vi "Water Tunnel Front Panel.vi"() -> ()   [LabVIEW 2019, in "Results.lvlib" / "Water Tunnel Results.lvclass"]
uses:
  Water Tunnel Results.lvclass
  Water Tunnel Results.lvclass/Water Tunnel Results.ctl
  Test Stands/Water Tunnel/Water Tunnel Test Stand.lvclass
panel:
  out "Water Flow Slide":dbl(slide) scale=0.0..100.0
  out "Wing Test":bool caption="Test"
  out "Wing Home":bool caption="Home"
  out "3-D Velocity":cluster{"Vx":dbl, "Vy":dbl, "Vz":dbl}
  out "Water flow":dbl format="%#.2f"
  out "Wing Angle of Attack":dbl(knob) scale=-45.0..45.0
  out "Probe depth":dbl(slide) scale=-100.0..100.0
  in  "Probe Z-Axis (Depth)":dbl
  in  "Wing Angle of Attack":dbl
  in  "Wing Test Position":bool
  in  "Wing Home Position":bool
  out "Wing Aligned?":bool=TRUE caption="Wing"
  out "Probe Aligned?":bool=TRUE caption="Probe"
  in  "Trav SetP":cluster{"Wx":dbl, "Wz":dbl, "Wa":dbl, "Pz":dbl}
  in  "Trav Probe Set?":bool caption="Probe Traverse"
  in  "Trav Wing Set?":bool caption="Wing Traverse"
  in  "Pump Load":dbl caption="Pump Load, %" step=10.0 format="%#.2f"
  out "p8":dbl format="%#.2f"
  out "p7":dbl format="%#.2f"
  out "p6":dbl format="%#.2f"
  out "p4":dbl format="%#.2f"
  out "p2":dbl format="%#.2f"
  out "p1":dbl format="%#.2f"
  out "p3":dbl format="%#.2f"
  out "p5":dbl format="%#.2f"
  out "Angle U":dbl format="%#.4f"
  out "Angle":dbl caption="Pitch" format="%#.2f"
  out "Data":waveform(dbl)[](graph) caption="Pressures"
  # "V"
  # "deg"
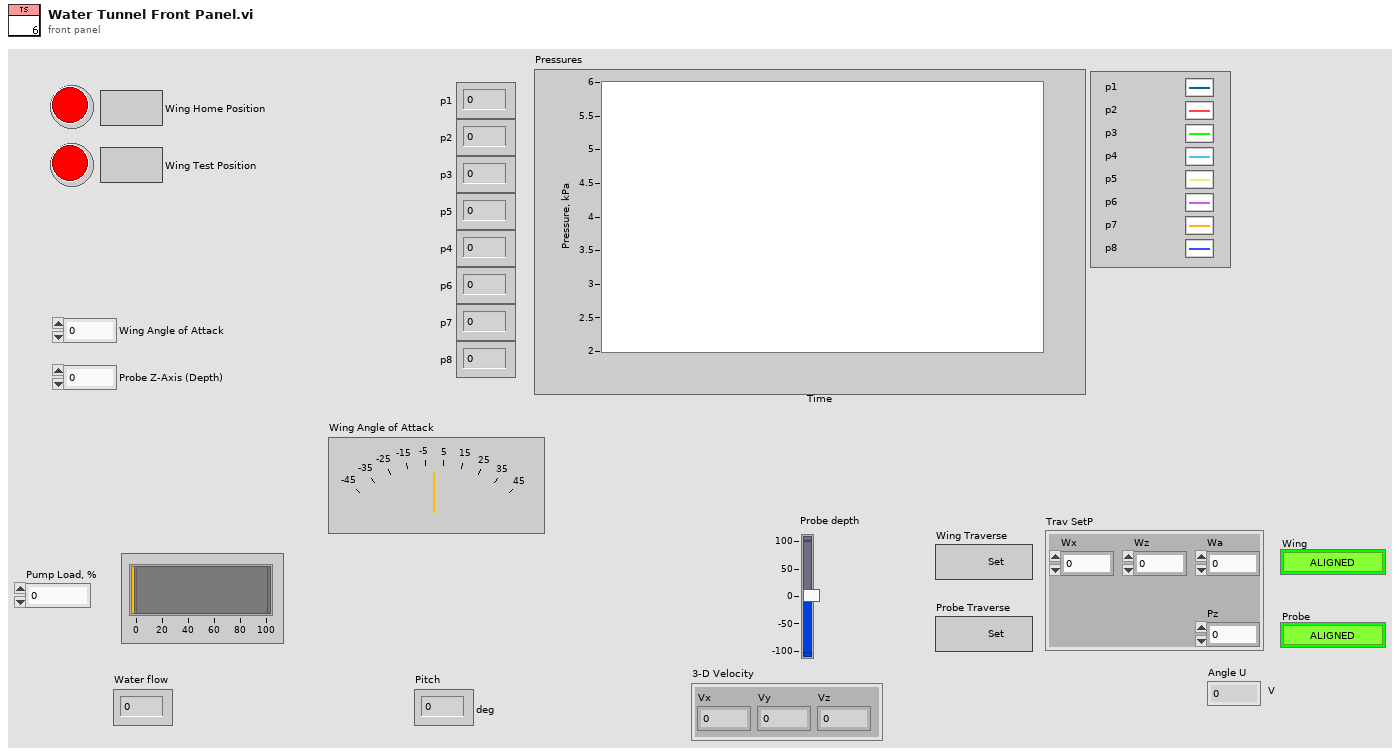
[diagram p1: front panel]
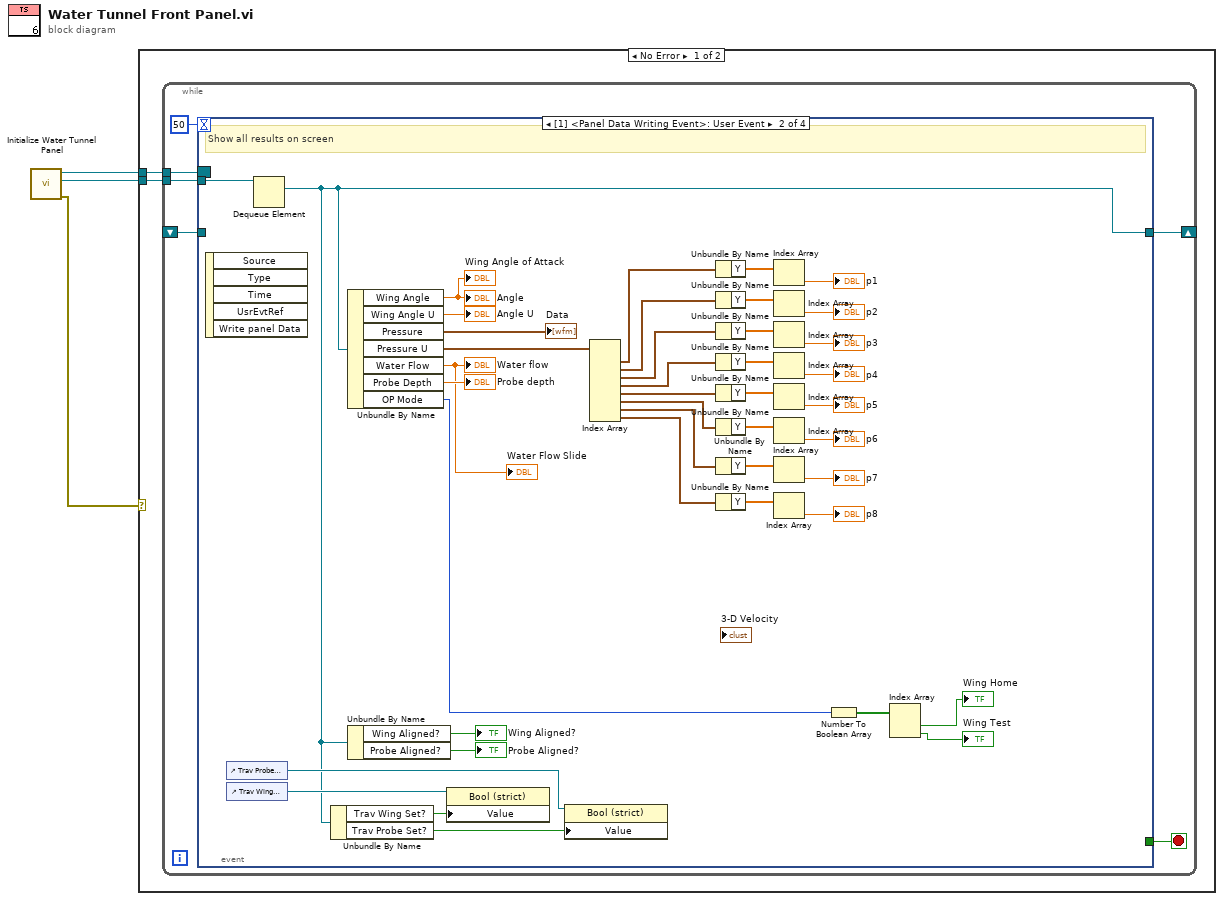
[diagram p0: block diagram]
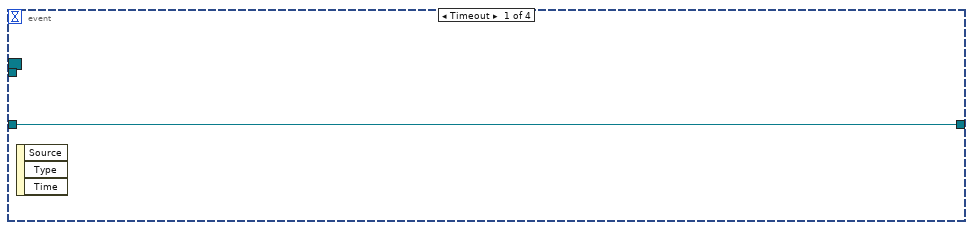
[diagram p2: hidden frame]
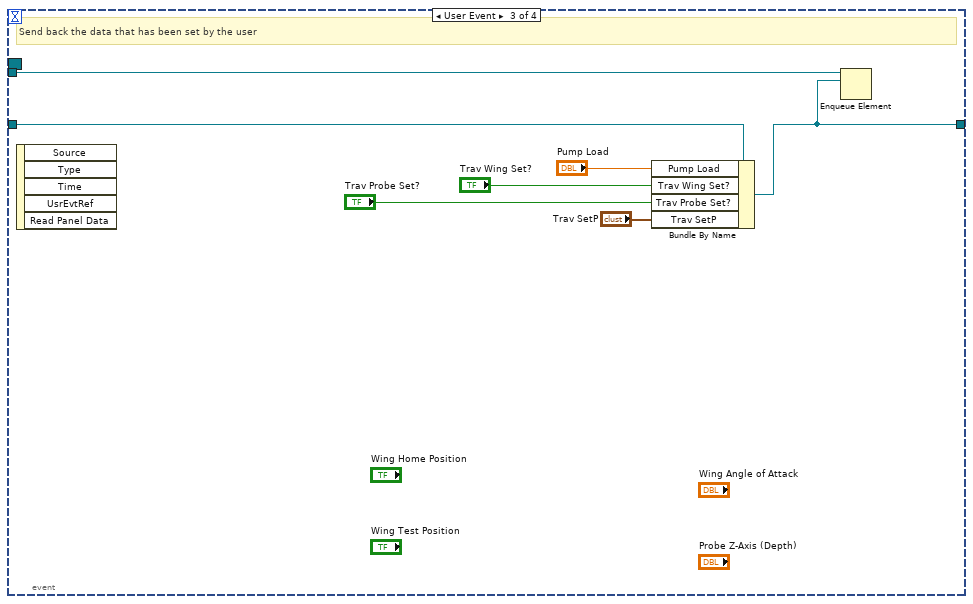
[diagram p3: hidden frame]
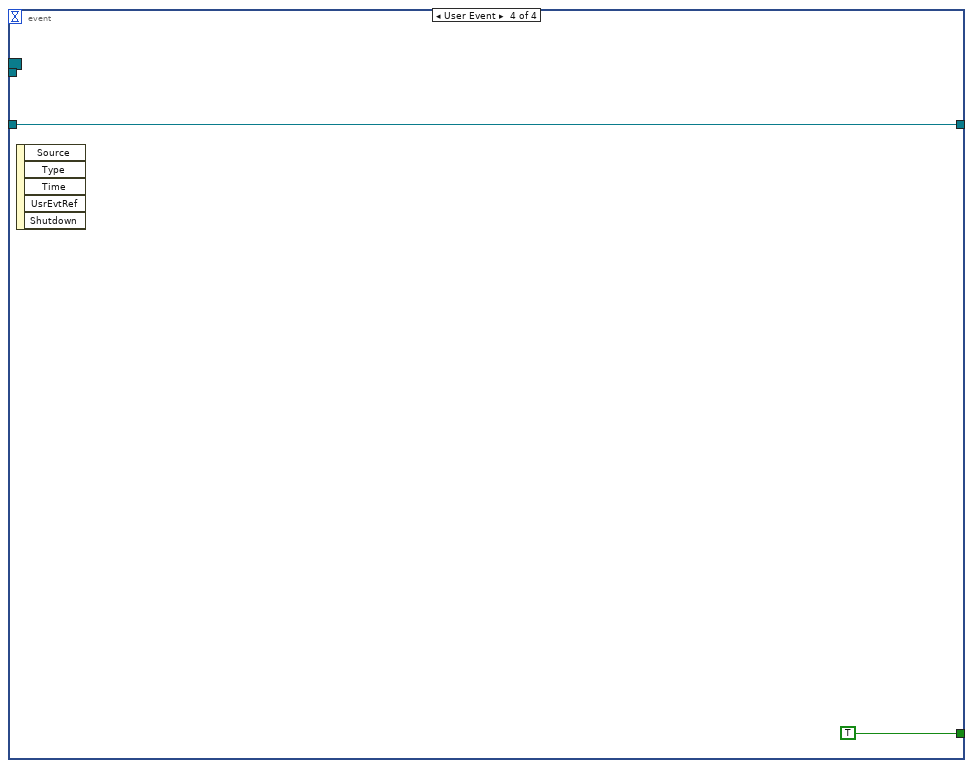
[diagram p4: hidden frame]
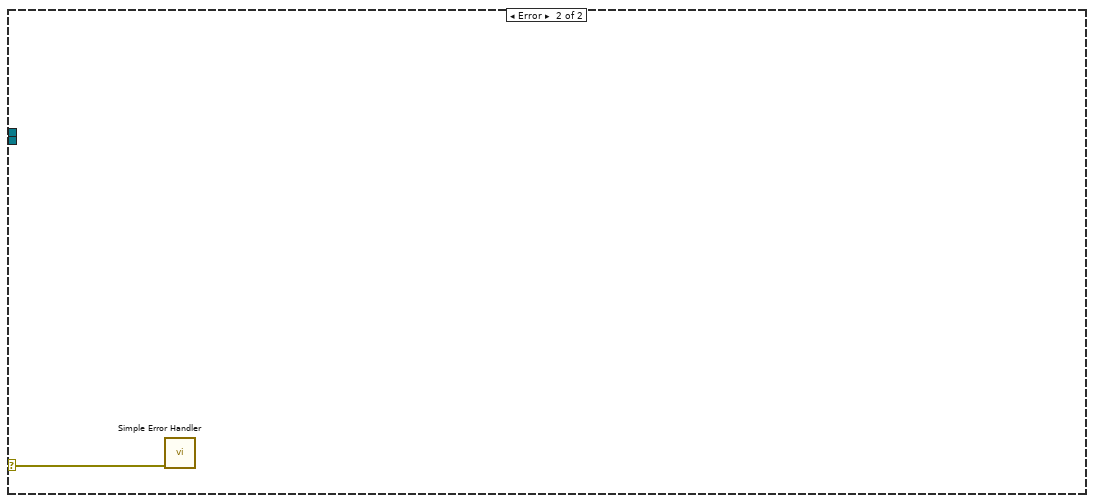
[diagram p5: hidden frame]
diagram:
  n1 = call "Initialize Water Tunnel Panel.vi"() -> ("error out"=w1:errorcluster, "Water Tunnel Results queue out"=w2:refnum<queue>, "Event Registration Refnum"=w3:refnum<event-registration>)  [unwired: 9 in]
  n2 = case shown="No Error" w1 {
    selector: w1 -> [_ w64]
    tunnel: w3 -> [w5 _]
    tunnel: w2 -> [w4 _]
    frame No Error {
      n3 = while {
        tunnel: w5 -> [w10]
        tunnel: w4 -> [w9]
        shift-right: [w7] -> _
        shift-left: _ -> [w6]
        stop <- w11 stop-if-true
        n4 = event shown="[1] <Panel Data Writing Event>: User Event" {
          selector: w10 -> [_ _ _ _]
          dyn-events: _ -> [_ _ _ _]
          timeout: 50 -> [_ _ _ _]
          tunnel: [_ _ _ TRUE] -> w11
          tunnel: w9 -> [_ w54 w61 _]
          tunnel: [w12 w23 w59 w62] -> w7
          tunnel: w6 -> [w12 _ w60 w62]
          event Timeout {
            n5 = event-data() -> ()  [unwired: 1 in, 3 out]
          }
          event User Event {
            # "Show all results on screen"
            n6 = event-data() -> ()  [unwired: 1 in, 5 out]
            n7 = control-ref of="Trav Probe Set?"() -> (w26:refnum<vi>)
            n8 = control-ref of="Trav Wing Set?"() -> (w27:refnum<vi>)
            n9 = Dequeue Element(queue=w54) -> (element=w23:refnum<class "Water Tunnel Results.lvclass">)  [unwired: 2 in, 3 out]
            n10 = Unbundle By Name(w23) -> ("Trav Wing Set?"=w25:bool, "Trav Probe Set?"=w24:bool)
            n11 = Unbundle By Name(w23) -> ("Wing Angle"=→"Angle" →"Wing Angle of Attack":dbl, "Wing Angle U"=→"Angle U":dbl, "Pressure"=→"Data":waveform(dbl)[], "Pressure U"=w29:waveform(dbl)[], "Water Flow"=→"Water flow" →"Water Flow Slide":dbl, "Probe Depth"=→"Probe depth":dbl, "OP Mode"=w17:u8)
            n12 = Unbundle By Name(w23) -> ("Wing Aligned?"=→"Wing Aligned?":bool, "Probe Aligned?"=→"Probe Aligned?":bool)
            n13 = property class="Bool (strict)"(reference=w27, "Value"=w25) -> ()  [unwired: 1 in, 2 out]
            n14 = property class="Bool (strict)"(reference=w26, "Value"=w24) -> ()  [unwired: 1 in, 2 out]
            n15 = Index Array(array=w29) -> (element #1=w53:waveform(dbl), element #2=w50:waveform(dbl), element #3=w47:waveform(dbl), element #4=w45:waveform(dbl), element #5=w43:waveform(dbl), element #6=w32:waveform(dbl), element #7=w31:waveform(dbl), element #8=w30:waveform(dbl))  [unwired: 8 in]
            n16 = Unbundle By Name(w53) -> ("Y"=w52:dbl[])
            n17 = Unbundle By Name(w50) -> ("Y"=w49:dbl[])
            n18 = Unbundle By Name(w47) -> ("Y"=w46:dbl[])
            n19 = Unbundle By Name(w45) -> ("Y"=w44:dbl[])
            n20 = Unbundle By Name(w43) -> ("Y"=w42:dbl[])
            n21 = Unbundle By Name(w32) -> ("Y"=w37:dbl[])
            n22 = Unbundle By Name(w31) -> ("Y"=w36:dbl[])
            n23 = Unbundle By Name(w30) -> ("Y"=w33:dbl[])
            n24 = Index Array(array=w52) -> (element=→"p1":dbl)  [unwired: 1 in]
            n25 = Index Array(array=w49) -> (element=→"p2":dbl)  [unwired: 1 in]
            n26 = Index Array(array=w46) -> (element=→"p3":dbl)  [unwired: 1 in]
            n27 = Index Array(array=w44) -> (element=→"p4":dbl)  [unwired: 1 in]
            n28 = Index Array(array=w42) -> (element=→"p5":dbl)  [unwired: 1 in]
            n29 = Index Array(array=w37) -> (element=→"p6":dbl)  [unwired: 1 in]
            n30 = Index Array(array=w36) -> (element=→"p7":dbl)  [unwired: 1 in]
            n31 = Index Array(array=w33) -> (element=→"p8":dbl)  [unwired: 1 in]
            n32 = Number To Boolean Array(number=w17) -> (Boolean array=w16:bool[])
            n33 = Index Array(array=w16) -> (element #1=→"Wing Home":bool, element #2=→"Wing Test":bool)  [unwired: 2 in]
          }
          event User Event {
            # "Send back the data that has been set by the user"
            n34 = event-data() -> ()  [unwired: 1 in, 5 out]
            n35 = Bundle By Name(cluster=w60, "Pump Load"="Pump Load", "Trav Wing Set?"="Trav Wing Set?", "Trav Probe Set?"="Trav Probe Set?", "Trav SetP"="Trav SetP") -> (w59:refnum<class "Water Tunnel Results.lvclass">)
            n36 = Enqueue Element(queue=w61, element=w59) -> ()  [unwired: 2 in, 3 out]
          }
          event User Event {
            n37 = event-data() -> ()  [unwired: 1 in, 5 out]
          }
        }
      }
    }
    frame Error {
      n38 = call <vilib>:"Simple Error Handler.vi"("error in (no error)"=w64) -> ()  [unwired: 4 in, 5 out]
    }
  }
